vi "snake.vi"() -> ()   [LabVIEW 2014]
doc: "Play the classic game snake!"
uses:
  xyplot.ctl
  Instance           1 13Saved   snake .vi
panel:
  out "Apples Eaten":i32
  in  "Max Apples":i32=20
  in  "Difficulty":u16(ring)=85 items=["Applications Engineer"=15, "Insane"=30, "Advanced"=50, "Intermediate"=85, "Noobie"=125]
  out "done":bool
  out "direction":dbl
  out "XY Graph":cluster{i32[], i32[]}[](graph)
  # "Snake"
  # "James McAndrew / October 2006"
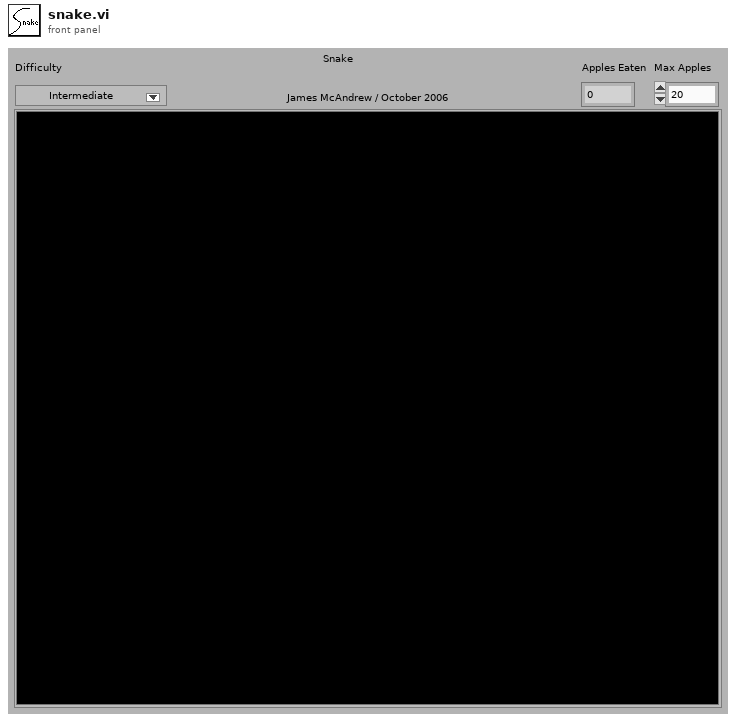
[diagram p1: front panel]
types:
  T1 = typedef "xyplot.ctl" = cluster{"X":i32[], "Y":i32[]}
  T2 = typedef "eventvkey.ctl" = enum16{"ASCII", "Enter", "Return", "Shift", "Ctrl", "Alt", "Cmd", "Opt", "Caps", "NumLock", "Clear", "Break", "Up", "Down", "Left", "Right", "Insert", "Delete", "Home", "End", "PageUp", "PageDown", "Escape", "Help", "Pause", "ScrollLock", "F1", "F2", "F3", "F4", "F5", "F6", "F7", "F8", "F9", "F10", "F11", "F12", "F13", "F14", "F15", "F16", "F17", "F18", "F19", "F20", "F21", "F22", "F23", "F24", "Play", "VolumeUp", "VolumeDown", "Mute", "Two Byte Char"}
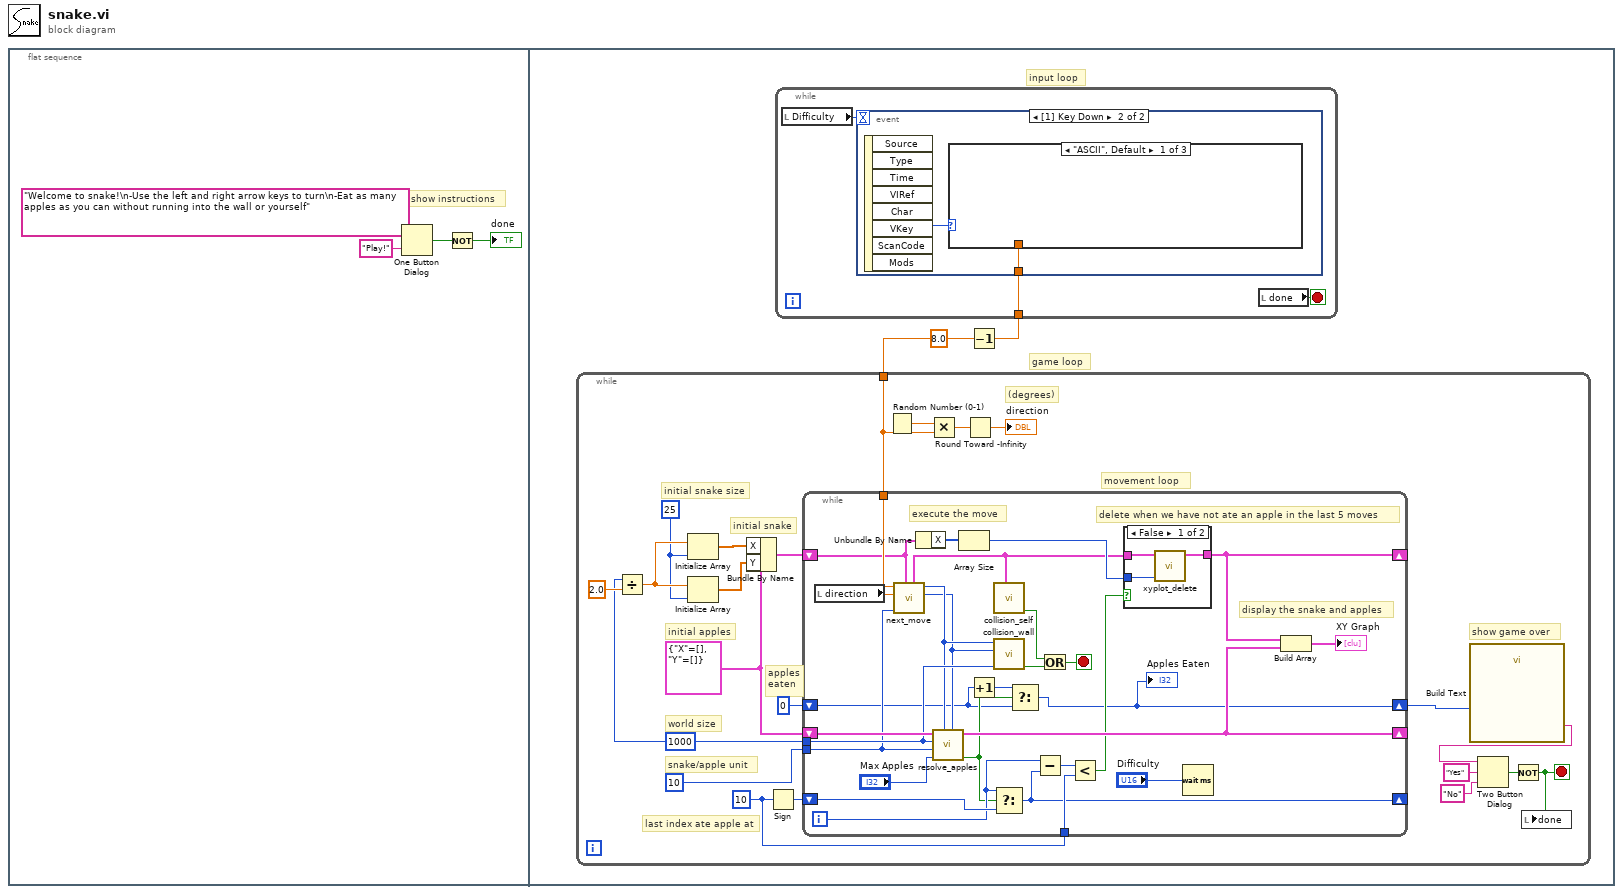
[diagram p0: block diagram]
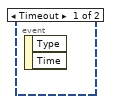
[diagram p2: hidden frame]
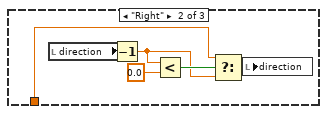
[diagram p3: hidden frame]
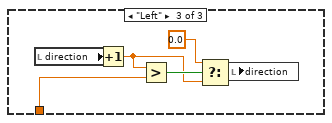
[diagram p4: hidden frame]
diagram:
  n1 = flat-sequence {
    frame #0 {
      # "show instructions"
      n2 = One Button Dialog(message="Welcome to snake!\n-Use the left and right arrow keys to turn\n-Eat as many apples as you can without running into the wall or yourself", button name ("OK")="Play!") -> (true=w4:bool)
      n3 = Not(x=w4) -> (.not. x?=→"done":bool)
    }
    frame #1 {
      w6 = 8.0
      # "game loop"
      # "input loop"
      n4 = while {
        tunnel: w6 -> [w30]
        stop <- w31 stop-if-true
        w26 = 10
        w33 = 25 ("y")
        w41 = T1 {"X"=[], "Y"=[]} ("XY Plot")
        w37 = 1000 ("y")
        # "apples\neaten"
        # "last index ate apple at"
        # "movement loop"
        # "initial snake size"
        # "show game over"
        # "world size"
        # "initial apples"
        # "snake/apple unit"
        # "(degrees)"
        # "initial snake"
        n5 = Divide(x=w37, y=2.0) -> (x/y=w36:dbl)
        n6 = Initialize Array(w36, w33) -> (w35:dbl[])
        n7 = Initialize Array(w36, w33) -> (w34:dbl[])
        n8 = Bundle By Name(cluster=w41, "X"=w35, "Y"=w34) -> (w40:T1)
        n9 = Sign(1:w26) -> (0:w27:i32)
        n10 = while {
          shift-right: [w56] -> _
          shift-left: w40 -> [w57]
          shift-right: [w69] -> _
          shift-left: w41 -> [w70]
          tunnel: 10 -> [w62]
          tunnel: w37 -> [w66]
          tunnel: w30 -> [w64]
          shift-right: [w50] -> _
          shift-left: w27 -> [w55]
          tunnel: w26 -> [w53]
          shift-right: [w48] -> w24
          shift-left: 0 -> [w47]
          i -> [w51]
          stop <- w73 stop-if-true
          # "display the snake and apples"
          # "delete when we have not ate an apple in the last 5 moves"
          # "execute the move"
          n11 = local read "direction"() -> (w63:dbl)
          n12 = call "next_move.vi"("Snake In"=w57, "Snake Unit"=w62, "Direction"=w63, "Direction max"=w64) -> ("Y"=w58:i32, "X"=w59:i32, "Snake Out"=w60:T1)  [unwired: 5 in]
          n13 = Unbundle By Name(w57) -> ("X"=w61:i32[])
          n14 = call "resolve_apples.vi"("Y"=w58, "X"=w59, "Max Apples"="Max Apples", "Apple Unit"=w62, "World Size"=w66, "Apples In"=w70) -> ("Ate Apple"=w49:bool, "Apples Out"=w69:T1)  [unwired: 4 in]
          n15 = Array Size(array=w61) -> (size(s)=w74:i32)
          n16 = Increment(x=w47) -> (x+1=w46:i32)
          n17 = call "collision_self.vi"("Snake Plot"=w60) -> ("Result"=w68:bool)  [unwired: 10 in]
          n18 = call "collision_wall.vi"("World Size"=w66, "Y"=w58, "X"=w59) -> ("Result"=w67:bool)  [unwired: 7 in]
          n19 = Select(t=w51, s=w49, f=w55) -> (s? t:f=w50:i32)
          n20 = Select(t=w46, s=w49, f=w47) -> (s? t:f=w48:i32)
          "Apples Eaten" <- w48
          n21 = Subtract(x=w51, y=w50) -> (x-y=w54:i32)
          n22 = Or(x=w68, y=w67) -> (x .or. y?=w73:bool)
          n23 = Less?(x=w54, y=w53) -> (x < y?=w52:bool)
          n24 = case shown="False" w52 {
            tunnel: [w77 w78] -> w56
            tunnel: w74 -> [w76 _]
            tunnel: w60 -> [w75 w78]
            frame False {
              n25 = call "xyplot_delete.vi"("index"=w76, "XY Plot Input"=w75) -> ("XY Plot Output"=w77:T1)  [unwired: 9 in]
            }
            frame True {
            }
          }
          n26 = Wait (ms)(milliseconds to wait="Difficulty") -> ()  [unwired: 1 out]
          n27 = Build Array(w56, w69) -> (→"XY Graph":T1[])
        }
        n28 = Random Number (0-1)() -> (number: 0 to 1=w39:dbl)
        n29 = Multiply(x=w39, y=w30) -> (x*y=w45:dbl)
        n30 = Round Toward -Infinity(1:w45) -> (0:→"direction":dbl)
        n31 = call "Build Text"("apples"=w24) -> ("Result"=w28:string)  [unwired: 13 in, 1 out]
        n32 = Two Button Dialog(message=w28, 1:"No" ("F button name (\"Cancel\")"), 2:"Yes" ("T button name (\"OK\")")) -> (T button?=w32:bool)
        n33 = Not(x=w32) -> (.not. x?=w31:bool)
        n34 = local write "done"(w31) -> ()
      }
      n35 = Decrement(x=w6) -> (x-1=w5:dbl)
      n36 = while {
        tunnel: w5 -> [w9]
        stop <- w8 stop-if-true
        n37 = local read "Difficulty"() -> (w7:u16)
        n38 = event shown="[1] Key Down" {
          selector: _ -> [_ _]
          dyn-events: _ -> [_ _]
          timeout: w7 -> [_ _]
          tunnel: w9 -> [_ w11]
          event Timeout {
            n39 = event-data() -> ()  [unwired: 1 in, 2 out]
          }
          event Key Down {
            n40 = event-data() -> ("VKey"=w10:T2)  [unwired: 1 in, 7 out]
            n41 = case shown="\"ASCII\", Default" w10 {
              tunnel: w11 -> [_ w12 w18]
              frame "ASCII", Default {
              }
              frame "Right" {
                n42 = local read "direction"() -> (w17:dbl)
                n43 = Decrement(x=w17) -> (x-1=w13:dbl)
                n44 = Less?(x=w13, y=0.0) -> (x < y?=w16:bool)
                n45 = Select(t=w12, s=w16, f=w13) -> (s? t:f=w14:dbl)
                n46 = local write "direction"(w14) -> ()
              }
              frame "Left" {
                n47 = local read "direction"() -> (w23:dbl)
                n48 = Increment(x=w23) -> (x+1=w19:dbl)
                n49 = Greater?(x=w19, y=w18) -> (0:w22:bool)
                n50 = Select(t=0.0 ("f"), s=w22, f=w19) -> (s? t:f=w21:dbl)
                n51 = local write "direction"(w21) -> ()
              }
            }
          }
        }
        n52 = local read "done"() -> (w8:bool)
      }
    }
  }
